vi "Receiver_Example - 2 Channel - Experiment_14.vi"() -> ()   [LabVIEW 2022 SP3]
panel:
  in  "stop":bool
  out "BER LP3":dbl
  out "BER HP3":dbl
  out "Inst. BER LP - CH1":dbl format="%#_4g"
  out "OutputHPCH0":i8[](array[numeric])
  out "BER 16QAM":dbl
  out "LP - CH0":dbl format="%#_4g"
  out "Numeric":i32
  out "HP - CH0":dbl format="%#_4g"
  out "x = 0?":bool
  out "iterationsIM":dbl
  in  "State":i32
  in  "Counter":dbl
  in  "Tab Control 3":enum32{"OFDM - 4QAM", "16QAM"}(tab)
  in  "Switch mode":bool
  in  "Tab Control":T1(tab)
  in  "USRP ControledParameters":T2={"Active Antenna"="RX2", "Gain (dB)"=10.0, "Carrier Frequency"=2400000000.0, "IQ Rate"=2000000.0, "Active channels"="0,1"} {"IQ Rate" format="%#_6p"; "Carrier Frequency" format="%#_6p"; "Gain (dB)" format="%#_6f"}
  in  "Device selection":refnum<k15>="RIO0"
  in  "Trigger level":dbl=0.01 format="%f"
  out "CH0":T3
  out "CH1":T3
  out "SIG valid? - CH1":bool
  out "SIG valid? - CH0":bool
  out "Frequency offset - CH1":dbl
  out "Frequency offset - CH0":dbl
  out "Coerced Parameters":T4={"IQ Rate"=100000.0, "Carrier  Freq."=100000.0, "Gain"=0.0} {"Gain" format="%#_6f"; "Carrier  Freq." format="%#_6p"; "IQ Rate" format="%#_6p"}
  out "Error out":errorcluster
  out "Inst. BER HP - CH0":dbl format="%#_4g"
  out "Acc. BER HP - CH0":dbl format="%#_4g"
  out "Acum. Err HP - CH0":dbl
  out "No. Bits HP - CH0":dbl
  out "Acc. BER LP - CH0":dbl format="%#_4g"
  out "Inst. BER - CH1":dbl format="%#_4g"
  out "Inst. BER LP - CH0":dbl format="%#_4g"
  out "No. Bits - CH1":dbl
  out "No. Bits LP - CH0":dbl
  out "Acum. Err - CH1":dbl
  out "Acum. Err LP - CH0":dbl
  in  "Record BER":bool
  in  "Refresh Button":bool
  out "Acc. BER - CH1":dbl format="%#_4g"
  in  "Boolean 2":bool
  in  "Expected message HP - CH0":string="Critical Dataaaaa\nCritical Dataaaaa\nCritical Dataaaaa\nCritical Dataaaaa\nCritical Dataaaaa"
  out "Expected message HP Detected CH0":string="Non Critical Data\nNon Critical Data\nNon Critical Data\nNon Critical Data\nNon Critical Data"
  in  "Boolean 3":bool
  in  "Boolean":bool
  out "Expected message HP Detected CH1":string="Non Critical Data\nNon Critical Data\nNon Critical Data\nNon Critical Data\nNon Critical Data"
  out "Expected message LP Detected CH0":string="Non Critical Data\nNon Critical Data\nNon Critical Data\nNon Critical Data\nNon Critical Data"
  in  "Expected message - CH1":string="Critical Dataaaaa\nCritical Dataaaaa\nCritical Dataaaaa\nCritical Dataaaaa\nCritical Dataaaaa"
  in  "Expected message LP - CH0":string="Non Critical Data\nNon Critical Data\nNon Critical Data\nNon Critical Data\nNon Critical Data"
  in  "Boolean 5":bool
  in  "Expected message LP - CH1":string="Non Critical Data\nNon Critical Data\nNon Critical Data\nNon Critical Data\nNon Critical Data"
  out "Expected message LP Detected CH1":string="Non Critical Data\nNon Critical Data\nNon Critical Data\nNon Critical Data\nNon Critical Data"
  in  "High-Power Window Size":dbl=15.0 format="%#_6p"
  in  "Low-Power Window Size - CH0":dbl=15.0 format="%#_6p"
  in  "Channel":bool
  in  "Expected message HP - CH0 2":string="Critical Dataaaaa\nCritical Dataaaaa\nCritical Dataaaaa\nCritical Dataaaaa\nCritical Dataaaaa\nNon Critical Data\nNon Critical Data\nNon Critical Data\nNon Critical Data\nNon Critical Data"
  in  "Tab Control 2":enum32{"1 Channel", "2 Channel"}(tab)
  in  "Save data 1 channel":bool
  out "Constellation Map 1 Channel":cdb[](graph)
  out "Low-Power BER - 1 Channel":dbl(graph)
  out "High-Power BER - 1 Channel":dbl(graph)
  out "High-Power Decoded message - 1 Channel":string
  out "Low-Power Decoded message - 1 Channel":string
  out "Low-Power Decoded message - CH0":string
  out "Decoded message - CH1":string
  out "Constellation Map 2 Channel":cluster{"Constellation":cdb[]}[](graph)
  out "Low-Power BER - 2 Channels":T5(graph)
  out "High-Power BER":T6(graph)
  out "High-Power Decoded message - CH0":string
  out "Low-Power Decoded message - CH1":string
  out "CH1 2":bool
  out "CH0 2":bool
  in  "Save data 2 channels":bool
  in  "Color Box 3":u32(colorbox)=11025761
  in  "Color Box 4":u32(colorbox)=7377308
  in  "Save data":bool
  out "Expected message  HP  Detected 2":string="Critical Dataaaaa\nCritical Dataaaaa\nCritical Dataaaaa\nCritical Dataaaaa\nCritical Dataaaaa"
  in  "Boolean 4":bool
  in  "High-Power Window Size 2":dbl=15.0 format="%#_6p"
  out "High-Power Instantaneous BER Graph 2":u8(slide) scale=0.0..100.0
  out "High-Power BER Graph 2":dbl(graph)
  out "No. Bits HP 2":dbl
  out "Acc. BER  HP 2":dbl format="%#_4g"
  out "Acum. Err HP 2":dbl
  out "Inst. BER HP 2":dbl format="%#_4g"
  in  "Expected message 2 HP 2":string="Critical Dataaaaa\nCritical Dataaaaa\nCritical Dataaaaa\nCritical Dataaaaa\nCritical Dataaaaa"
  out "High-Power Decoded Message 2":string
  in  "Record BER 2":bool
  out "Constellation Map 2":cdb[](graph)
  out "Frequency offset 2":dbl
  out "SIG valid? 2":bool
  in  "Refresh Button 2":bool
  out "Error out 2":errorcluster
  in  "error in (no error)":errorcluster
  # "OFDM Superposition Coded Receiver"
  # "Superposition coded\n(criticality-aware)"
  # "Single stream\n(criticality-agnostic)"
  # "1 Channel"
  # "2 Channel"
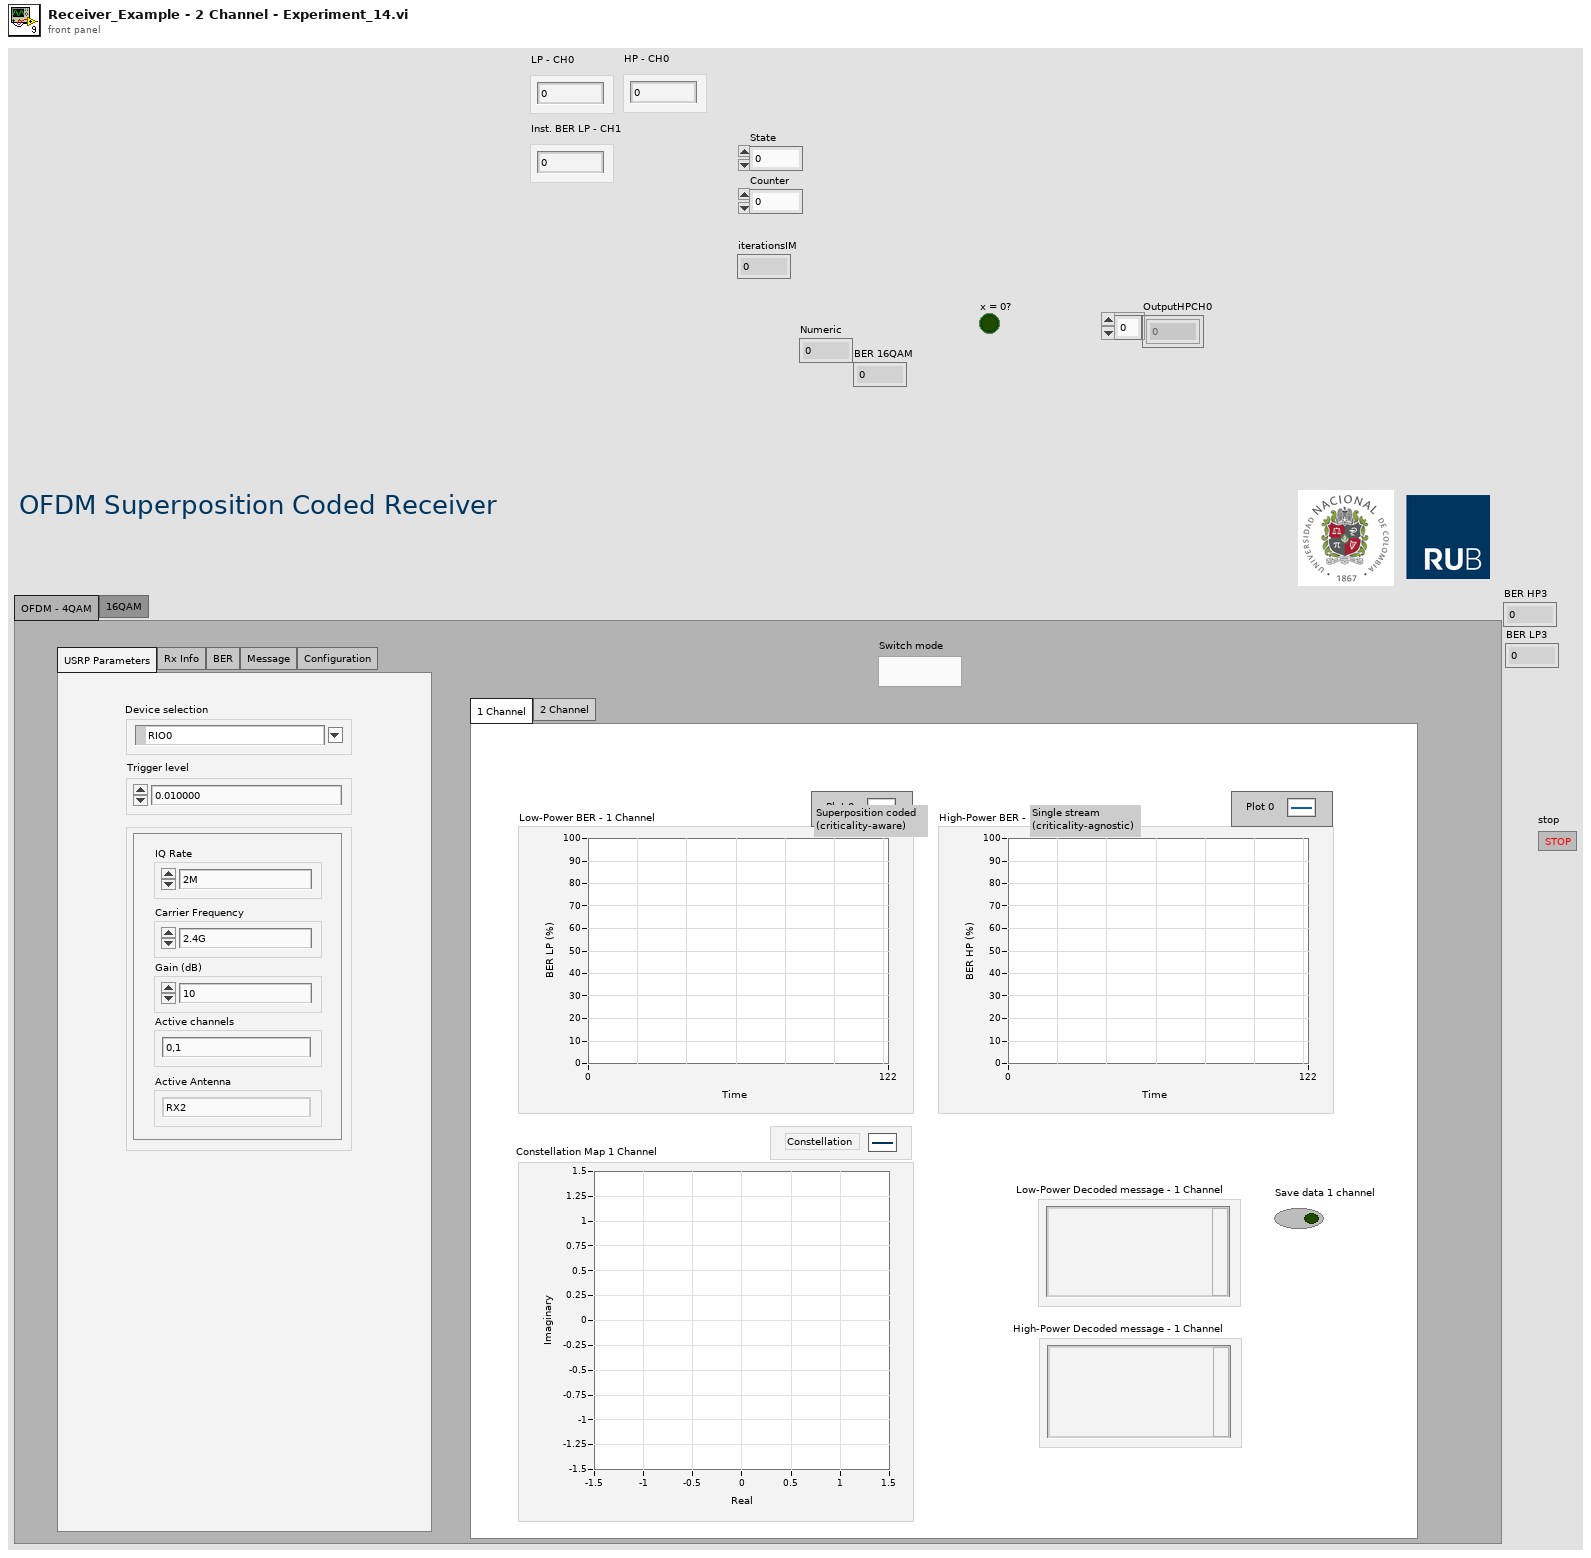
[diagram p1: front panel]
types:
  T1 = enum32{"USRP Parameters", "Rx Info", "BER", "Message", "Configuration"}
  T2 = cluster{"Active Antenna":string, "Gain (dB)":dbl, "Carrier Frequency":dbl, "IQ Rate":dbl, "Active channels":string}
  T3 = cluster{"Modulation type":enum16{"QPSK(4QAM)", "64QAM", "16QAM", "BPSK"}, "BCC rate (k/n)":enum16{"1/2", "2/3", "3/4"}}
  T4 = cluster{"IQ Rate":dbl, "Carrier  Freq.":dbl, "Gain":dbl}
  T5 = cluster{"Graph Instantaneous BER":dbl, "Graph Instantaneous BER":dbl, "Graph Instantaneous BER":dbl}
  T6 = cluster{"Graph Instantaneous BER":dbl, "Graph Instantaneous BER":dbl, "Inst. BER - CH1":dbl}
  T7 = enum16{"open", "replace", "create", "open or create", "replace or create", "replace or create with confirmation"}
  T8 = cluster{"coerced IQ rate":dbl, "coerced carrier frequency":dbl, "coerced gain":dbl}
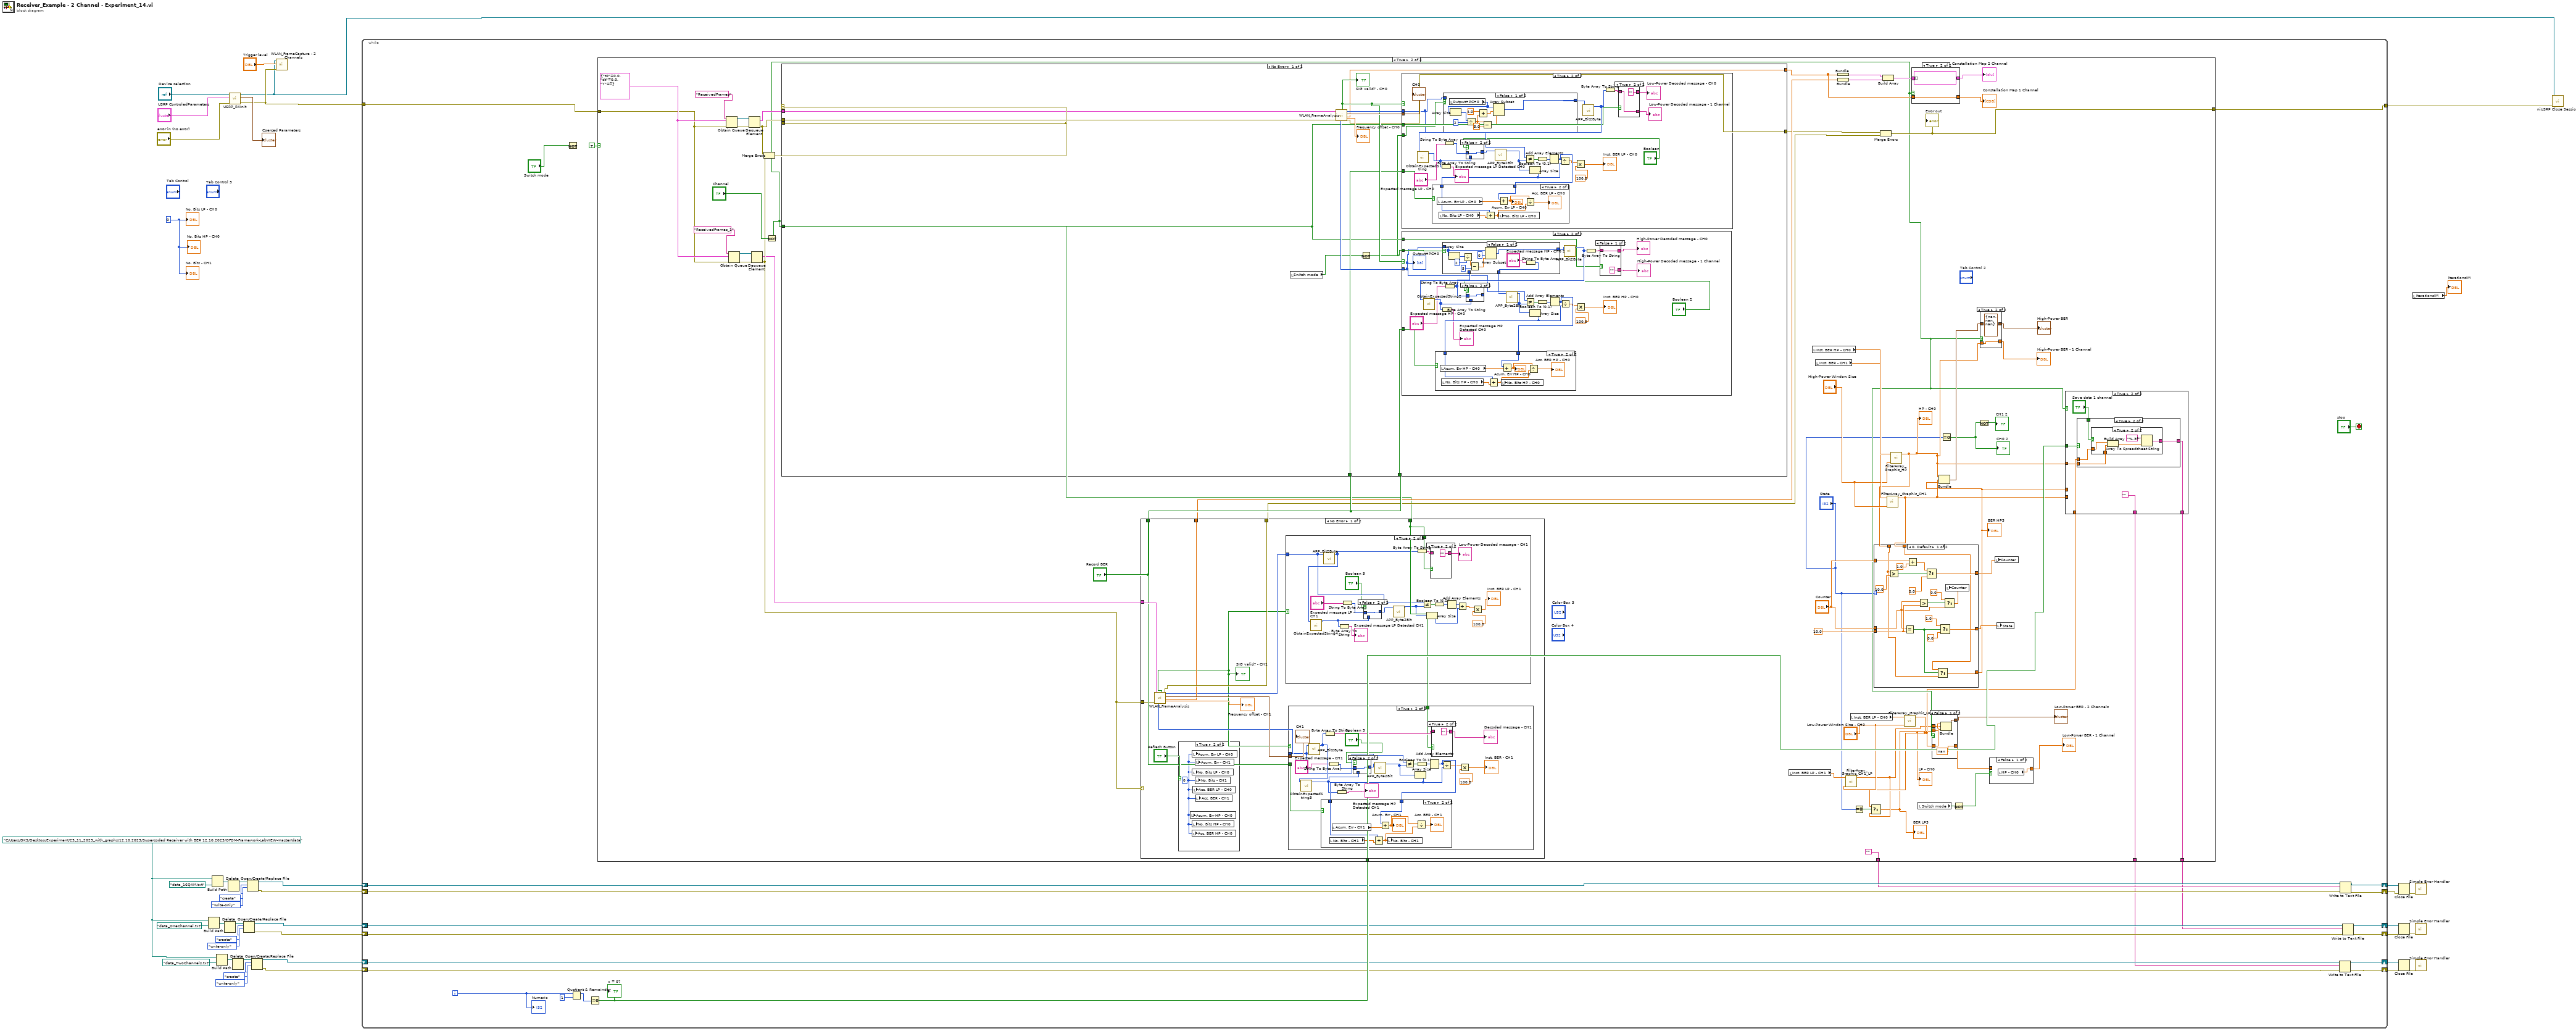
[diagram p0: block diagram]
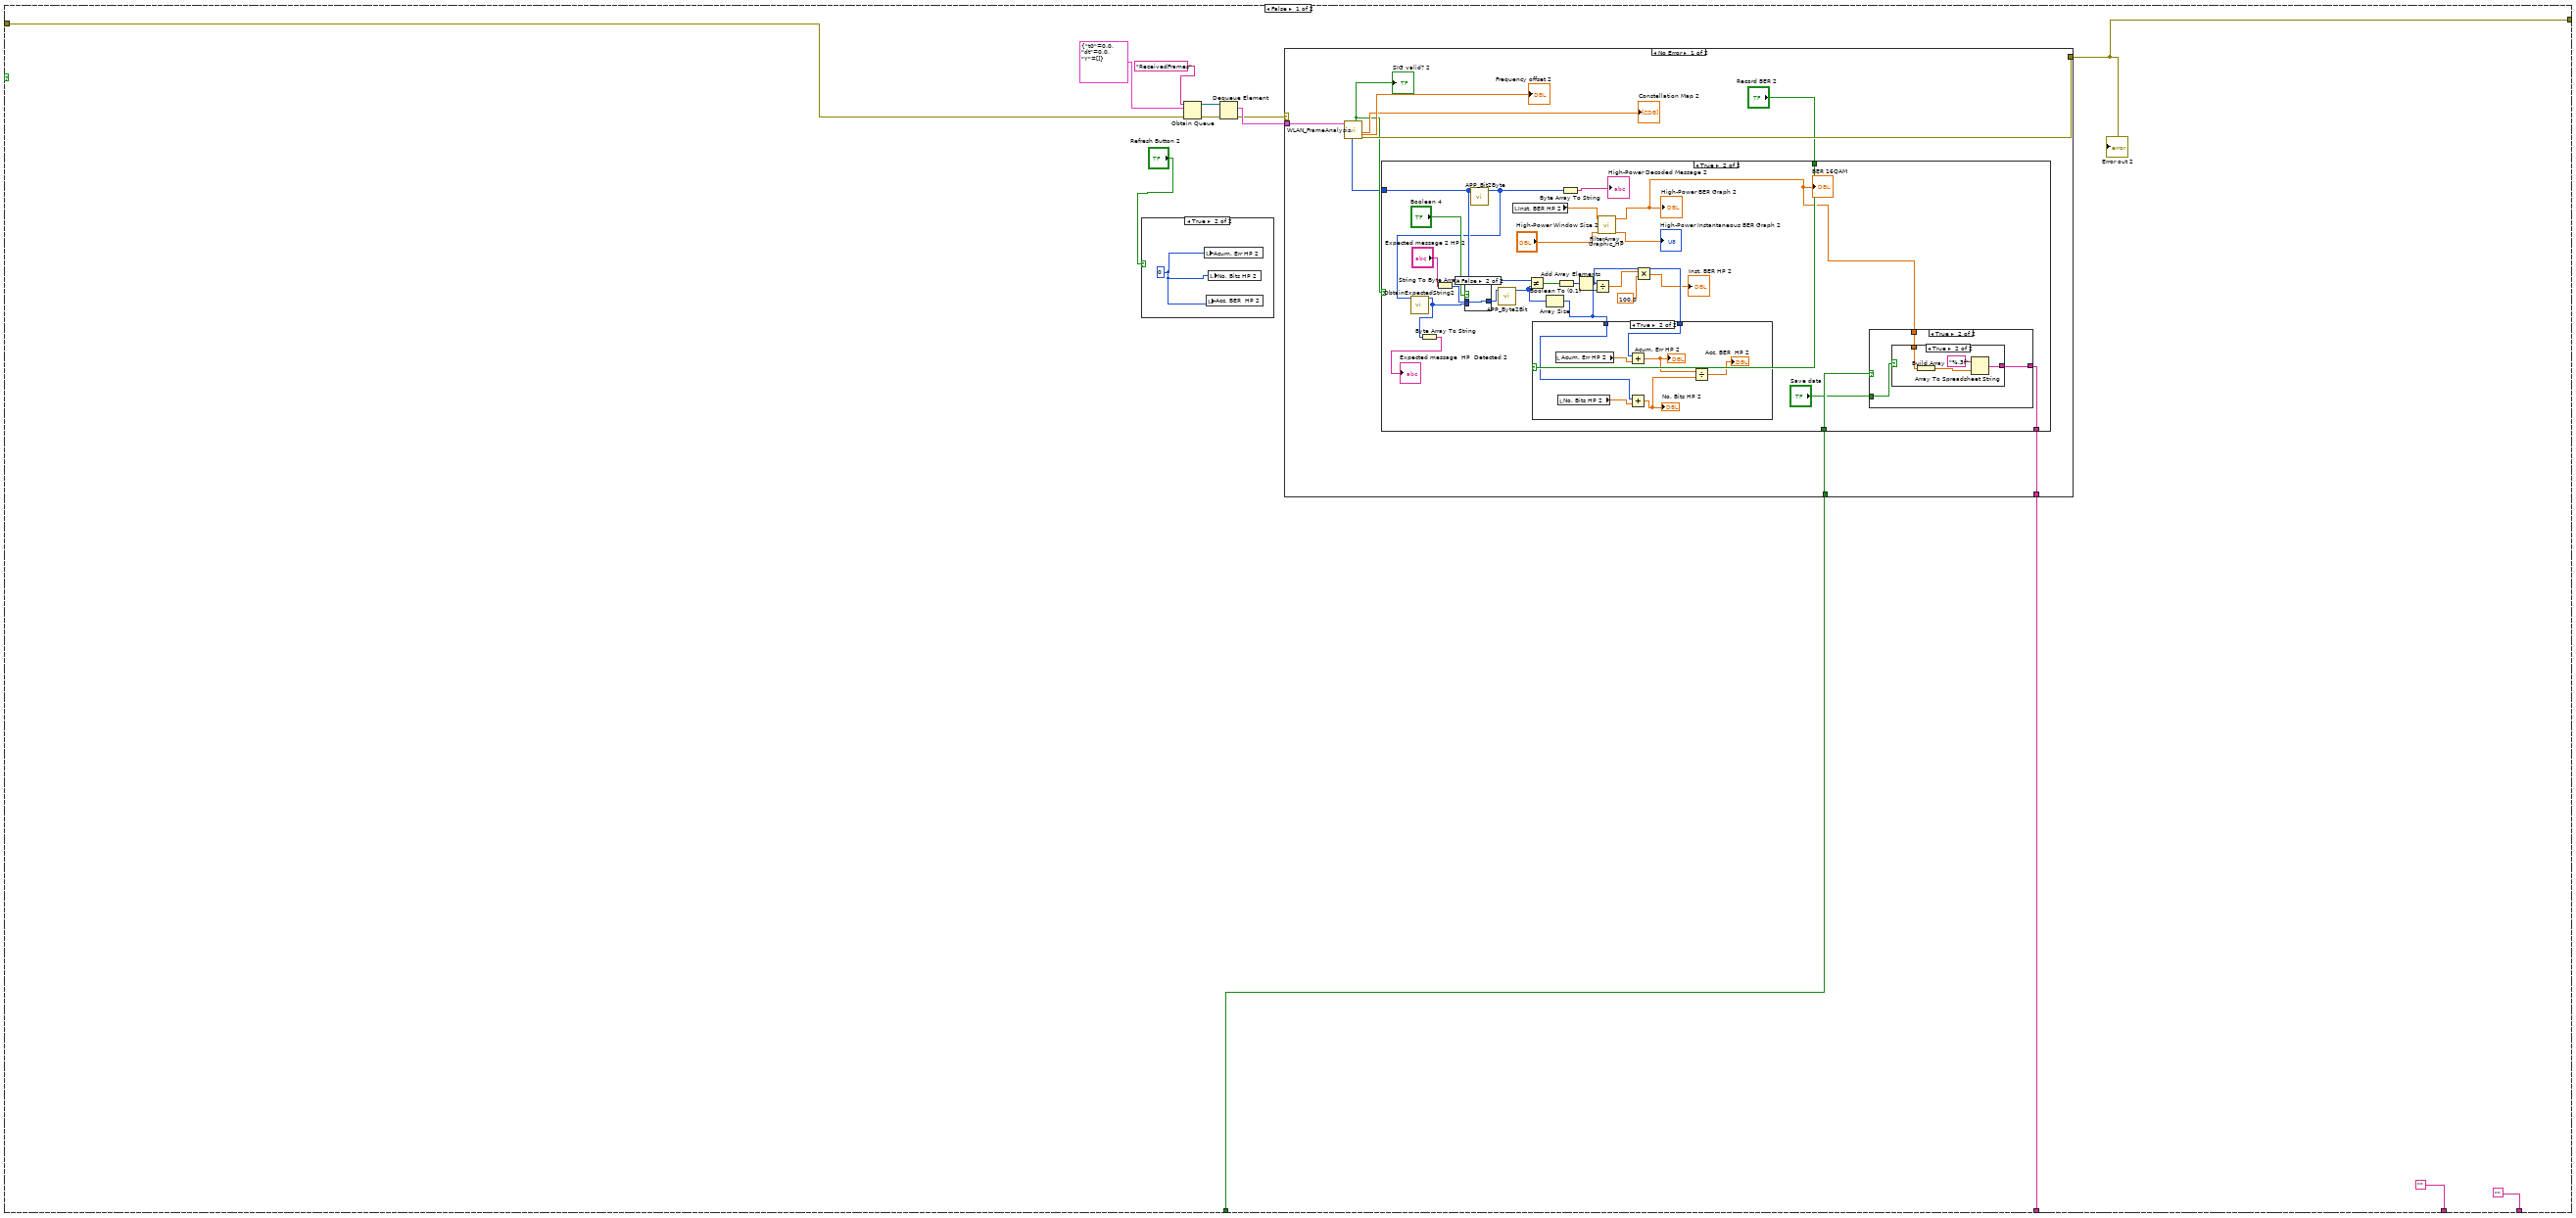
[diagram p2: hidden frame]
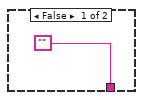
[diagram p4: hidden frame]
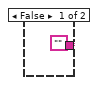
[diagram p5: hidden frame]
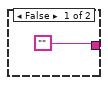
[diagram p6: hidden frame]
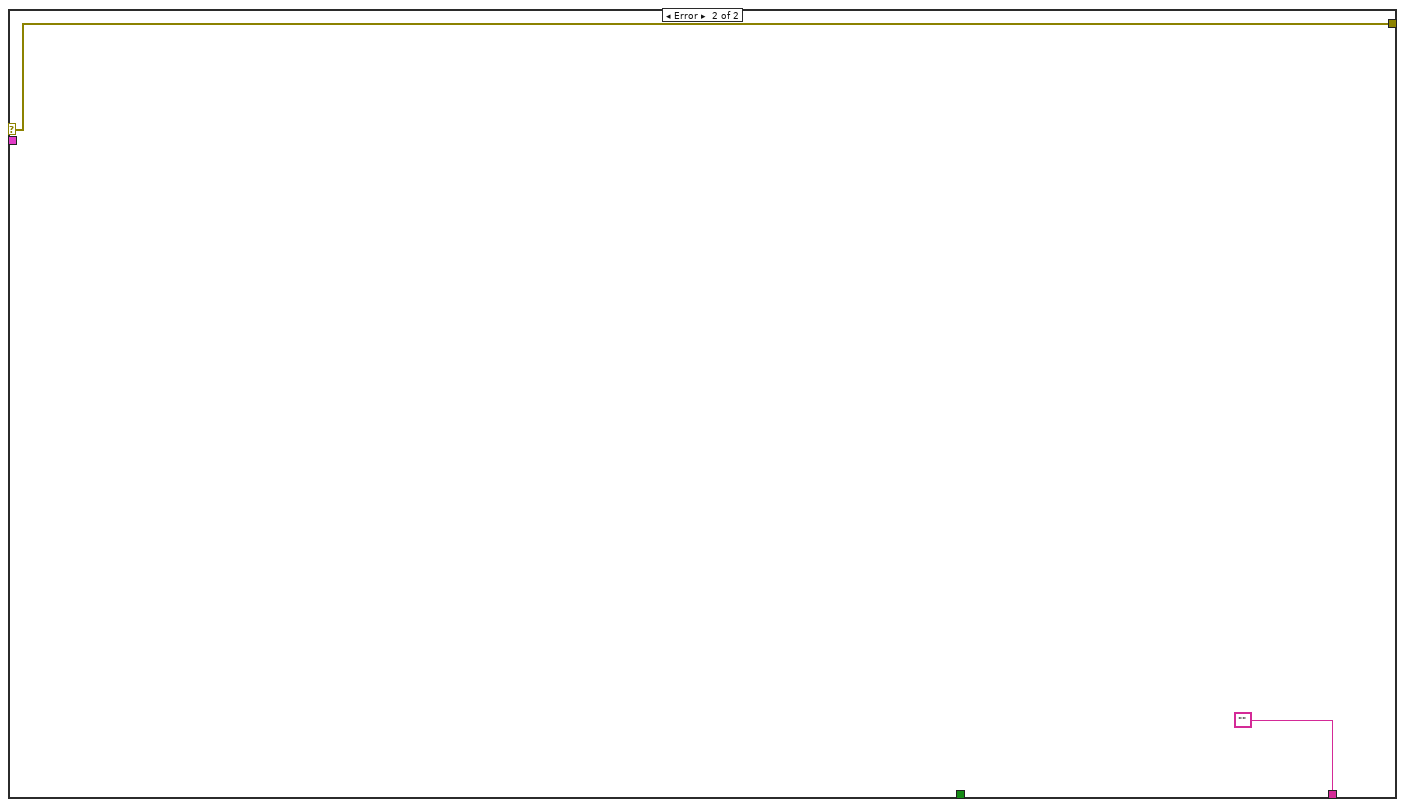
[diagram p9: hidden frame]
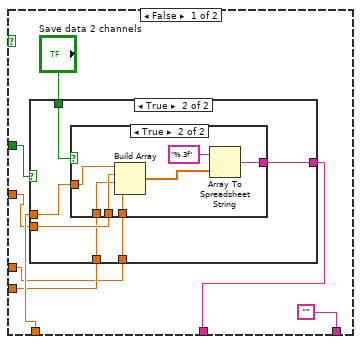
[diagram p11: hidden frame]
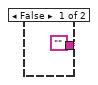
[diagram p12: hidden frame]
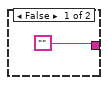
[diagram p13: hidden frame]
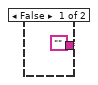
[diagram p14: hidden frame]
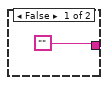
[diagram p15: hidden frame]
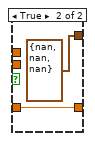
[diagram p16: hidden frame]
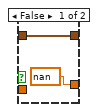
[diagram p17: hidden frame]
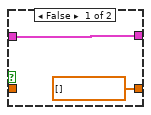
[diagram p18: hidden frame]
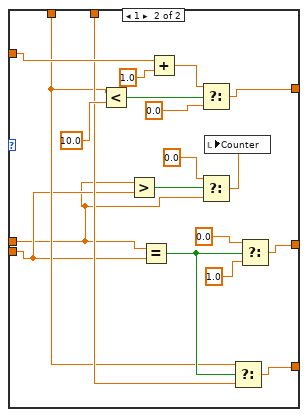
[diagram p19: hidden frame]
diagram:
  w11 = path "C:/Users/DKS/Desktop/Experiment/23_11_2023_with_graphs/12.10.2023/Supercoded Receiver with BER 12.10.2023/OFDM-Framework-LabVIEW-master/data"
  w33 = 0
  n1 = Build Path(base path=w11, name or relative path=path "data_OneChannel.txt" ("default name")) -> (appended path=w21:path)
  n2 = Build Path(base path=w11, name or relative path=path "data_16QAM.txt" ("default name")) -> (appended path=w31:path)
  n3 = Build Path(base path=w11, name or relative path=path "data_TwoChannels.txt" ("default name")) -> (appended path=w16:path)
  n4 = Delete(path (use dialog)=w21) -> (deleted path=w20:path)  [unwired: 4 in, 2 out]
  n5 = Delete(path (use dialog)=w31) -> (deleted path=w30:path)  [unwired: 4 in, 2 out]
  n6 = call "USRP_RXInit.vi"("device names"="Device selection", "USRP ControledParameters"="USRP ControledParameters", "error in (no error)"="error in (no error)") -> ("session handle out"=w36:refnum<k15>, "USRP CoercedParamters"=→"Coerced Parameters":T8, "error out"=w39:errorcluster)  [unwired: 5 in]
  n7 = Delete(path (use dialog)=w16) -> (deleted path=w15:path)  [unwired: 4 in, 2 out]
  n8 = Open/Create/Replace File(file path (use dialog)=w20, operation (0:open)=T7."create", access (0:read/write)=enum16{"read/write", "read-only", "write-only"}."write-only") -> (refnum out=w8:refnum<file>, error out=w7:errorcluster)  [unwired: 1 in, 3 out]
  n9 = Open/Create/Replace File(file path (use dialog)=w30, operation (0:open)=T7."create", access (0:read/write)=enum16{"read/write", "read-only", "write-only"}."write-only") -> (refnum out=w24:refnum<file>, error out=w25:errorcluster)  [unwired: 1 in, 3 out]
  n10 = Open/Create/Replace File(file path (use dialog)=w15, operation (0:open)=T7."create", access (0:read/write)=enum16{"read/write", "read-only", "write-only"}."write-only") -> (refnum out=w6:refnum<file>, error out=w5:errorcluster)  [unwired: 1 in, 3 out]
  n11 = call "WLAN_FrameCapture - 2 Channels.vi"("error in (no error)"=w39, "Trigger level"="Trigger level", "session handle"=w36) -> ()  [unwired: 8 in]
  n12 = while {
    tunnel: w39 -> [w65]
    tunnel: [w64] -> w37
    shift-right: [w60] -> w23
    shift-left: w25 -> [w58]
    shift-right: [w59] -> w22
    shift-left: w24 -> [w57]
    shift-right: [w54] -> w4
    shift-left: w8 -> [w55]
    shift-right: [w52] -> w3
    shift-left: w7 -> [w53]
    shift-right: [w48] -> w2
    shift-left: w6 -> [w51]
    shift-right: [w49] -> w1
    shift-left: w5 -> [w50]
    i -> [w45]
    stop <- "stop" stop-if-true
    n13 = Not(x="Switch mode") -> ()  [unwired: 1 out]
    n14 = Quotient & Remainder(x=w45, y=1) -> (x-y*floor(x/y)=w62:i32)  [unwired: 1 out]
    n15 = Equal To 0?(x=w62) -> (x = 0?=w61:bool)
    "x = 0?" <- w61
    n16 = case shown="True" TRUE {
      tunnel: w65 -> [w71 w157]
      tunnel: [w70 w156] -> w64
      tunnel: w61 -> [w69 w152]
      tunnel: [w68 ""] -> w56
      tunnel: ["" w151] -> w47
      tunnel: ["" w149] -> w46
      frame False {
        n17 = case shown="True" "Refresh Button 2" {
          frame False {
          }
          frame True {
            w79 = 0
            n18 = local write "Acum. Err HP 2"(w79) -> ()
            n19 = local write "Acc. BER  HP 2"(w79) -> ()
            n20 = local write "No. Bits HP 2"(w79) -> ()
          }
        }
        n21 = Obtain Queue(name (unnamed)="ReceivedFrames", element data type=cluster{"t0":dbl, "dt":dbl, "Y":cdb[]} {"t0"=0.0, "dt"=0.0, "Y"=[]} ("data"), error in (no error)=w71) -> (queue out=w72:refnum<queue>, error out=w75:errorcluster)  [unwired: 2 in, 1 out]
        n22 = Dequeue Element(queue=w72, error in (no error)=w75) -> (element=w74:cluster{"t0":dbl, "dt":dbl, "Y":cdb[]}, error out=w73:errorcluster)  [unwired: 1 in, 2 out]
        n23 = case shown="No Error" w73 {
          selector: w73 -> [_ w134]
          tunnel: w74 -> [w87 _]
          tunnel: [w88 w134] -> w70
          tunnel: w69 -> [w81 _]
          tunnel: [w80 ""] -> w68
          frame No Error {
            n24 = call "WLAN_FrameAnalysis.vi"("input cluster"=w87) -> ("error out"=w88:errorcluster, "Constellation"=→"Constellation Map 2":cdb[], "Frequency offset"=→"Frequency offset 2":dbl, "SIG valid?"=w83:bool, "outputbitsHP"=w82:i8[])  [unwired: 4 in, 2 out]
            "SIG valid? 2" <- w83
            n25 = case shown="True" w83 {
              tunnel: "Record BER 2" -> [_ w108]
              tunnel: w82 -> [_ w103]
              tunnel: w81 -> [_ w93]
              tunnel: ["" w91] -> w80
              frame False {
              }
              frame True {
                n26 = String To Byte Array(string="Expected message 2 HP 2") -> (unsigned byte array=w101:u8[])
                n27 = call "APP_Bit2Byte.vi"("input bit stream"=w103) -> ("output byte stream"=w97:u8[])  [unwired: 10 in]
                n28 = call "ObtainExpectedString2.vi"("Array"=w97) -> ("detectedMessage"=w99:i8[])  [unwired: 9 in]
                n29 = Byte Array To String(unsigned byte array=w99) -> (string=→"Expected message  HP  Detected 2":string)
                n30 = case shown="False" "Boolean 4" {
                  tunnel: [w124 w125] -> w102
                  tunnel: w101 -> [_ w125]
                  tunnel: w99 -> [w124 _]
                  frame True {
                  }
                  frame False {
                  }
                }
                n31 = call "APP_Byte2Bit.vi"("input byte stream"=w102) -> ("output bit stream"=w104:i8[])  [unwired: 10 in]
                n32 = local read "Inst. BER HP 2"() -> (w107:dbl)
                n33 = Not Equal?(x=w103, y=w104) -> (x != y?=w112:bool[])
                n34 = Array Size(array=w104) -> (size(s)=w109:i32)
                n35 = Boolean To (0,1)(Boolean=w112) -> (0, 1=w111:i16[])
                n36 = Byte Array To String(unsigned byte array=w97) -> (string=→"High-Power Decoded Message 2":string)
                n37 = Add Array Elements(numeric array=w111) -> (sum=w110:i16)
                n38 = case shown="True" w108 {
                  tunnel: w110 -> [_ w131]
                  tunnel: w109 -> [_ w126]
                  frame False {
                  }
                  frame True {
                    n39 = local read "Acum. Err HP 2"() -> (w132:dbl)
                    n40 = local read "No. Bits HP 2"() -> (w128:dbl)
                    n41 = Add(x=w131, y=w132) -> (x+y=w130:dbl)
                    "Acum. Err HP 2" <- w130
                    n42 = Add(x=w126, y=w128) -> (x+y=w127:dbl)
                    "No. Bits HP 2" <- w127
                    n43 = Divide(x=w130, y=w127) -> (x/y=→"Acc. BER  HP 2":dbl)
                  }
                }
                n44 = Divide(x=w110, y=w109) -> (x/y=w96:dbl)
                n45 = call "FilterArray_Graphic_HP.vi"("Window Size"="High-Power Window Size 2", "Instantaneous BER"=w107) -> ("Slide Bar"=→"High-Power Instantaneous BER Graph 2":dbl, "Graph Instantaneous BER"=w90:dbl)  [unwired: 4 in]
                "High-Power BER Graph 2" <- w90
                "BER 16QAM" <- w90
                n46 = Multiply(x=w96, y=100.0) -> (x*y=→"Inst. BER HP 2":dbl)
                n47 = case shown="True" w93 {
                  tunnel: ["" w118] -> w91
                  tunnel: w90 -> [_ w117]
                  tunnel: "Save data" -> [_ w116]
                  frame False {
                  }
                  frame True {
                    n48 = case shown="True" w116 {
                      tunnel: ["" w121] -> w118
                      tunnel: w117 -> [_ w120]
                      frame False {
                      }
                      frame True {
                        n49 = Build Array(w120) -> (w123:dbl[])
                        n50 = Array To Spreadsheet String(array=w123, 3:"%.3f") -> (spreadsheet string=w121:string)  [unwired: 1 out]
                      }
                    }
                  }
                }
              }
            }
          }
          frame Error {
          }
        }
        "Error out 2" <- w70
      }
      frame True {
        w192 = cluster{"t0":dbl, "dt":dbl, "Y":cdb[]} {"t0"=0.0, "dt"=0.0, "Y"=[]} ("data")
        n51 = Obtain Queue(name (unnamed)="ReceivedFrames", element data type=w192, error in (no error)=w157) -> (queue out=w158:refnum<queue>, error out=w160:errorcluster)  [unwired: 2 in, 1 out]
        n52 = Obtain Queue(name (unnamed)="ReceivedFrames_1", element data type=w192, error in (no error)=w157) -> (queue out=w162:refnum<queue>, error out=w163:errorcluster)  [unwired: 2 in, 1 out]
        n53 = Dequeue Element(queue=w158, error in (no error)=w160) -> (element=w159:cluster{"t0":dbl, "dt":dbl, "Y":cdb[]}, error out=w166:errorcluster)  [unwired: 1 in, 2 out]
        n54 = Dequeue Element(queue=w162, error in (no error)=w163) -> (element=w168:cluster{"t0":dbl, "dt":dbl, "Y":cdb[]}, error out=w172:errorcluster)  [unwired: 1 in, 2 out]
        n55 = Merge Errors(w166, w172) -> (w165:errorcluster)
        n56 = Not(x="Channel") -> (.not. x?=w153:bool)
        n57 = case shown="No Error" w165 {
          tunnel: w159 -> [w368 _]
          tunnel: w165 -> [_ w468]
          tunnel: w166 -> [w365 _]
          tunnel: [w364 dbl[] []] -> w183
          tunnel: [w363 w468] -> w169
          tunnel: "Record BER" -> [w362 _]
          tunnel: "Record BER" -> [w361 _]
          tunnel: w153 -> [w360 _]
          frame No Error {
            n58 = local read "Switch mode"() -> (w359:bool)
            n59 = call "WLAN_FrameAnalysis.vi"("error in (no error)"=w365, "input cluster"=w368) -> ("error out"=w363:errorcluster, "Constellation"=w364:cdb[], "Modulation parameter"=w369:T3, "output bits"=w370:i8[], "Frequency offset"=→"Frequency offset - CH0":dbl, "SIG valid?"=w366:bool, "outputbitsHP"=w367:i8[])  [unwired: 3 in]
            "SIG valid? - CH0" <- w366
            n60 = Not(x=w359) -> (.not. x?=w358:bool)
            n61 = case shown="True" w366 {
              tunnel: w370 -> [_ w423]
              tunnel: w369 -> [_ w443]
              tunnel: w361 -> [_ w440]
              tunnel: w360 -> [_ w426]
              tunnel: w358 -> [_ w424]
              frame False {
              }
              frame True {
                n62 = case shown="False" w424 {
                  tunnel: w423 -> [_ w453]
                  tunnel: [w451 w453] -> w425
                  frame False {
                    n63 = local read "OutputHPCH0"() -> (w450:i8[])
                    n64 = Array Size(array=w450) -> (size(s)=w449:i32)
                    n65 = Divide(x=w449, y=2) -> (x/y=w446:dbl)
                    n66 = Add(x=4.0, y=w446) -> (x+y=w448:dbl)
                    n67 = Subtract(x=w446, y=5.0) -> (x-y=w444:dbl)
                    n68 = Array Subset(array=w450, index=w448, length=w444) -> (w451:i8[])
                  }
                  frame True {
                  }
                }
                n69 = String To Byte Array(string="Expected message LP - CH0") -> (unsigned byte array=w433:u8[])
                n70 = call "APP_Bit2Byte.vi"("input bit stream"=w425) -> ("output byte stream"=w432:u8[])  [unwired: 10 in]
                n71 = call "ObtainExpectedString.vi"("Array"=w432) -> ("detectedMessage"=w431:i8[])  [unwired: 9 in]
                n72 = Byte Array To String(unsigned byte array=w431) -> (string=→"Expected message LP Detected CH0":string)
                n73 = case shown="False" "Boolean" {
                  tunnel: [w458 w459] -> w435
                  tunnel: w433 -> [_ w459]
                  tunnel: w431 -> [w458 _]
                  frame True {
                  }
                  frame False {
                  }
                }
                n74 = call "APP_Byte2Bit.vi"("input byte stream"=w435) -> ("output bit stream"=w434:i8[])  [unwired: 10 in]
                n75 = Not Equal?(x=w423, y=w434) -> (x != y?=w441:bool[])
                n76 = Array Size(array=w434) -> (size(s)=w439:i32)
                n77 = Boolean To (0,1)(Boolean=w441) -> (0, 1=w442:i16[])
                n78 = Add Array Elements(numeric array=w442) -> (sum=w438:i16)
                n79 = case shown="True" w440 {
                  tunnel: w439 -> [_ w465]
                  tunnel: w438 -> [_ w463]
                  frame False {
                  }
                  frame True {
                    n80 = local read "Acum. Err LP - CH0"() -> (w464:dbl)
                    n81 = local read "No. Bits LP - CH0"() -> (w466:dbl)
                    n82 = Add(x=w465, y=w466) -> (x+y=w462:dbl)
                    n83 = Add(x=w463, y=w464) -> (x+y=w461:dbl)
                    "Acum. Err LP - CH0" <- w461
                    n84 = local write "No. Bits LP - CH0"(w462) -> ()
                    n85 = Divide(x=w461, y=w462) -> (x/y=→"Acc. BER LP - CH0":dbl)
                  }
                }
                n86 = Divide(x=w438, y=w439) -> (x/y=w437:dbl)
                n87 = Multiply(x=w437, y=100.0) -> (x*y=→"Inst. BER LP - CH0":dbl)
                n88 = Byte Array To String(unsigned byte array=w432) -> (string=w429:string)
                n89 = case shown="True" w426 {
                  tunnel: w429 -> [w455 w457]
                  tunnel: ["" ("string") w457] -> w428
                  tunnel: [w455 "" ("string")] -> w427
                  frame False {
                  }
                  frame True {
                  }
                }
                "Low-Power Decoded message - CH0" <- w427
                "Low-Power Decoded message - 1 Channel" <- w428
                "CH0" <- w443
              }
            }
            n90 = case shown="True" w366 {
              tunnel: w367 -> [_ w376]
              tunnel: w362 -> [_ w392]
              tunnel: w360 -> [_ w381]
              tunnel: w358 -> [_ w379]
              frame False {
              }
              frame True {
                n91 = String To Byte Array(string="Expected message HP - CH0") -> (unsigned byte array=w378:u8[])
                n92 = case shown="False" w379 {
                  tunnel: w376 -> [w402 w406]
                  tunnel: [w403 w406] -> w380
                  tunnel: [w395 w405] -> w375
                  tunnel: w378 -> [_ w405]
                  frame False {
                    n93 = Array Size(array=w402) -> (size(s)=w399:i32)
                    n94 = Divide(x=w399, y=2) -> (x/y=w398:dbl)
                    n95 = Subtract(x=w398, y=5) -> (x-y=w400:dbl)
                    n96 = Array Subset(array=w402, index=0, length=w400) -> (w403:i8[])
                    n97 = String To Byte Array(string="Expected message HP - CH0 2") -> (unsigned byte array=w395:u8[])
                  }
                  frame True {
                  }
                }
                n98 = call "APP_Byte2Bit.vi"("input byte stream"=w375) -> ("output bit stream"=w377:i8[])  [unwired: 10 in]
                n99 = Not Equal?(x=w376, y=w377) -> (x != y?=w393:bool[])
                n100 = Array Size(array=w377) -> (size(s)=w391:i32)
                n101 = Boolean To (0,1)(Boolean=w393) -> (0, 1=w394:i16[])
                n102 = Add Array Elements(numeric array=w394) -> (sum=w390:i16)
                n103 = case shown="True" w392 {
                  tunnel: w391 -> [_ w418]
                  tunnel: w390 -> [_ w416]
                  frame False {
                  }
                  frame True {
                    n104 = local read "Acum. Err HP - CH0"() -> (w417:dbl)
                    n105 = local read "No. Bits HP - CH0"() -> (w419:dbl)
                    n106 = Add(x=w418, y=w419) -> (x+y=w415:dbl)
                    n107 = local write "No. Bits HP - CH0"(w415) -> ()
                    n108 = Add(x=w416, y=w417) -> (x+y=w414:dbl)
                    "Acum. Err HP - CH0" <- w414
                    n109 = Divide(x=w414, y=w415) -> (x/y=→"Acc. BER HP - CH0":dbl)
                  }
                }
                n110 = Divide(x=w390, y=w391) -> (x/y=w389:dbl)
                n111 = call "APP_Bit2Byte.vi"("input bit stream"=w380) -> ("output byte stream"=w387:u8[])  [unwired: 10 in]
                n112 = call "ObtainExpectedString2.vi"("Array"=w387) -> ("detectedMessage"=w386:i8[])  [unwired: 9 in]
                n113 = Byte Array To String(unsigned byte array=w386) -> (string=→"Expected message HP Detected CH0":string)
                n114 = case shown="False" "Boolean 2" {
                  tunnel: [w411 w412] -> _
                  tunnel: w378 -> [_ w412]
                  tunnel: w386 -> [w411 _]
                  frame True {
                  }
                  frame False {
                  }
                }
                n115 = Multiply(x=w389, y=100.0) -> (x*y=→"Inst. BER HP - CH0":dbl)
                n116 = Byte Array To String(unsigned byte array=w387) -> (string=w382:string)
                n117 = case shown="False" w381 {
                  tunnel: w382 -> [w408 w410]
                  tunnel: ["" ("string") w410] -> w383
                  tunnel: [w408 "" ("string")] -> w384
                  frame False {
                  }
                  frame True {
                  }
                }
                "High-Power Decoded message - CH0" <- w384
                "High-Power Decoded message - 1 Channel" <- w383
                "OutputHPCH0" <- w376
              }
            }
          }
          frame Error {
          }
        }
        n118 = case shown="No Error" w172 {
          tunnel: w168 -> [w295 _]
          tunnel: "Record BER" -> [w294 _]
          tunnel: [w293 w357] -> w170
          tunnel: [w292 dbl[] []] -> w171
          tunnel: w172 -> [w291 w357]
          tunnel: w153 -> [w288 _]
          frame No Error {
            n119 = call "WLAN_FrameAnalysis.vi"("error in (no error)"=w291, "input cluster"=w295) -> ("error out"=w293:errorcluster, "Constellation"=w292:cdb[], "Modulation parameter"=w298:T3, "output bits"=w290:i8[], "Frequency offset"=→"Frequency offset - CH1":dbl, "SIG valid?"=w289:bool, "outputbitsHP"=w296:i8[])  [unwired: 3 in]
            "SIG valid? - CH1" <- w289
            n120 = case shown="True" "Refresh Button" {
              frame False {
              }
              frame True {
                w323 = 0
                n121 = local write "Acum. Err HP - CH0"(w323) -> ()
                n122 = local write "Acc. BER HP - CH0"(w323) -> ()
                n123 = local write "Acum. Err LP - CH0"(w323) -> ()
                n124 = local write "No. Bits LP - CH0"(w323) -> ()
                n125 = local write "No. Bits HP - CH0"(w323) -> ()
                n126 = local write "Acc. BER LP - CH0"(w323) -> ()
                n127 = local write "Acum. Err - CH1"(w323) -> ()
                n128 = local write "No. Bits - CH1"(w323) -> ()
                n129 = local write "Acc. BER - CH1"(w323) -> ()
              }
            }
            n130 = case shown="True" w289 {
              tunnel: w290 -> [_ w301]
              tunnel: w288 -> [_ w316]
              frame False {
              }
              frame True {
                n131 = call "APP_Bit2Byte.vi"("input bit stream"=w301) -> ("output byte stream"=w311:u8[])  [unwired: 10 in]
                n132 = call "ObtainExpectedString4.vi"("Array"=w311) -> ("detectedMessage"=w312:i8[])  [unwired: 9 in]
                n133 = Byte Array To String(unsigned byte array=w312) -> (string=→"Expected message LP Detected CH1":string)
                n134 = String To Byte Array(string="Expected message LP - CH1") -> (unsigned byte array=w315:u8[])
                n135 = case shown="False" "Boolean 5" {
                  tunnel: [w319 w320] -> w310
                  tunnel: w315 -> [_ w320]
                  tunnel: w312 -> [w319 _]
                  frame True {
                  }
                  frame False {
                  }
                }
                n136 = call "APP_Byte2Bit.vi"("input byte stream"=w310) -> ("output bit stream"=w302:i8[])  [unwired: 10 in]
                n137 = Byte Array To String(unsigned byte array=w311) -> (string=w318:string)
                n138 = Not Equal?(x=w301, y=w302) -> (x != y?=w308:bool[])
                n139 = Array Size(array=w302) -> (size(s)=w307:i32)
                n140 = case shown="True" w316 {
                  tunnel: w318 -> [w321 _]
                  tunnel: [w321 "" ("string")] -> w317
                  frame False {
                  }
                  frame True {
                  }
                }
                "Low-Power Decoded message - CH1" <- w317
                n141 = Boolean To (0,1)(Boolean=w308) -> (0, 1=w309:i16[])
                n142 = Add Array Elements(numeric array=w309) -> (sum=w306:i16)
                n143 = Divide(x=w306, y=w307) -> (x/y=w305:dbl)
                n144 = Multiply(x=w305, y=100.0) -> (x*y=→"Inst. BER LP - CH1":dbl)
              }
            }
            n145 = case shown="True" w289 {
              tunnel: w296 -> [_ w332]
              tunnel: w298 -> [_ w344]
              tunnel: w294 -> [_ w330]
              tunnel: w288 -> [_ w327]
              frame False {
              }
              frame True {
                n146 = call "APP_Bit2Byte.vi"("input bit stream"=w332) -> ("output byte stream"=w334:u8[])  [unwired: 10 in]
                n147 = call "ObtainExpectedString3.vi"("Array"=w334) -> ("detectedMessage"=w333:i8[])  [unwired: 9 in]
                n148 = Byte Array To String(unsigned byte array=w334) -> (string=w328:string)
                n149 = String To Byte Array(string="Expected message - CH1") -> (unsigned byte array=w335:u8[])
                n150 = Byte Array To String(unsigned byte array=w333) -> (string=→"Expected message HP Detected CH1":string)
                n151 = case shown="False" "Boolean 3" {
                  tunnel: [w347 w348] -> w337
                  tunnel: w335 -> [_ w348]
                  tunnel: w333 -> [w347 _]
                  frame True {
                  }
                  frame False {
                  }
                }
                n152 = call "APP_Byte2Bit.vi"("input byte stream"=w337) -> ("output bit stream"=w336:i8[])  [unwired: 10 in]
                n153 = Not Equal?(x=w332, y=w336) -> (x != y?=w342:bool[])
                n154 = Array Size(array=w336) -> (size(s)=w341:i32)
                n155 = Boolean To (0,1)(Boolean=w342) -> (0, 1=w343:i16[])
                n156 = Add Array Elements(numeric array=w343) -> (sum=w340:i16)
                n157 = case shown="True" w330 {
                  tunnel: w341 -> [_ w354]
                  tunnel: w340 -> [_ w352]
                  frame False {
                  }
                  frame True {
                    n158 = local read "No. Bits - CH1"() -> (w355:dbl)
                    n159 = local read "Acum. Err - CH1"() -> (w353:dbl)
                    n160 = Add(x=w354, y=w355) -> (x+y=w351:dbl)
                    n161 = Add(x=w352, y=w353) -> (x+y=w350:dbl)
                    "Acum. Err - CH1" <- w350
                    n162 = local write "No. Bits - CH1"(w351) -> ()
                    n163 = Divide(x=w350, y=w351) -> (x/y=→"Acc. BER - CH1":dbl)
                  }
                }
                n164 = case shown="True" w327 {
                  tunnel: w328 -> [w345 _]
                  tunnel: [w345 "" ("string")] -> w329
                  frame False {
                  }
                  frame True {
                  }
                }
                "Decoded message - CH1" <- w329
                n165 = Divide(x=w340, y=w341) -> (x/y=w338:dbl)
                n166 = Multiply(x=w338, y=100.0) -> (x*y=→"Inst. BER - CH1":dbl)
                "CH1" <- w344
              }
            }
          }
          frame Error {
          }
        }
        n167 = local read "Inst. BER LP - CH1"() -> (w141:dbl)
        n168 = local read "Inst. BER HP - CH0"() -> (w188:dbl)
        n169 = local read "Inst. BER - CH1"() -> (w179:dbl)
        n170 = Bundle("Constellation"=w183) -> (w182:cluster{"Constellation":cdb[]})  [unwired: 1 in]
        n171 = Bundle("Constellation"=w171) -> (w167:cluster{"Constellation":cdb[]})  [unwired: 1 in]
        n172 = call "FilterArray_Graphic_CH1_LP.vi"("Window Size"="Low-Power Window Size - CH0", "Instantaneous BER"=w141) -> ("Graph Instantaneous BER"=w136:dbl)  [unwired: 4 in, 1 out]
        n173 = local read "Inst. BER LP - CH0"() -> (w154:dbl)
        n174 = Equal To 0?(x="State") -> (x = 0?=w139:bool)
        n175 = Merge Errors(w169, w170) -> (w156:errorcluster)
        "Error out" <- w156
        n176 = Build Array(w182, w167) -> (w185:cluster{"Constellation":cdb[]}[])
        n177 = call "FilterArray_Graphic_CH1.vi"("Window Size"="High-Power Window Size", "Instantaneous BER"=w179) -> ("Graph Instantaneous BER"=w150:dbl)  [unwired: 4 in, 1 out]
        n178 = call "FilterArray_Graphic_HP.vi"("Window Size"="High-Power Window Size", "Instantaneous BER"=w188) -> ("Graph Instantaneous BER"=w147:dbl)  [unwired: 4 in, 1 out]
        "HP - CH0" <- w147
        n179 = case shown="0, Default" "State" {
          tunnel: "Counter" -> [w256 w276]
          tunnel: [w263 w279] -> w175
          tunnel: "Counter" -> [w251 w269]
          tunnel: [w260 w278] -> w176
          tunnel: [w258 w277] -> w148
          tunnel: w147 -> [w257 w274]
          tunnel: w150 -> [w255 w275]
          tunnel: 10.0 ("y") -> [w254 w270]
          frame 0, Default {
            n180 = Greater?(x=w257, y=10.0) -> (0:w264:bool)
            n181 = Equal?(x=w251, y=w254) -> (x = y?=w259:bool)
            n182 = Add(x=w256, y=1.0) -> (x+y=w266:dbl)
            n183 = Greater?(x=w251, y=w254) -> (0:w253:bool)
            n184 = Select(t=w266, s=w264, f=0.0) -> (s? t:f=w263:dbl)
            n185 = Select(t=w255, s=w259, f=w257) -> (s? t:f=w258:dbl)
            n186 = Select(t=1.0, s=w259, f=0.0) -> (s? t:f=w260:dbl)
            n187 = Select(t=0.0, s=w253, f=w251) -> (s? t:f=w250:dbl)
            n188 = local write "Counter"(w250) -> ()
          }
          frame 1 {
            n189 = Less?(x=w274, y=10.0) -> (x < y?=w280:bool)
            n190 = Greater?(x=w269, y=w270) -> (0:w272:bool)
            n191 = Equal?(x=w269, y=w270) -> (x = y?=w282:bool)
            n192 = Add(x=w276, y=1.0) -> (x+y=w286:dbl)
            n193 = Select(t=w286, s=w280, f=0.0) -> (s? t:f=w279:dbl)
            n194 = Select(t=0.0, s=w272, f=w269) -> (s? t:f=w273:dbl)
            n195 = local write "Counter"(w273) -> ()
            n196 = Select(t=w274, s=w282, f=w275) -> (s? t:f=w277:dbl)
            n197 = Select(t=0.0, s=w282, f=1.0) -> (s? t:f=w278:dbl)
          }
        }
        "BER HP3" <- w148
        n198 = call "FilterArray_Graphic_LP.vi"("Window Size"="Low-Power Window Size - CH0", "Instantaneous BER"=w154) -> ("Graph Instantaneous BER"=w137:dbl)  [unwired: 4 in, 1 out]
        "LP - CH0" <- w137
        n199 = Select(t=w137, s=w139, f=w136) -> (s? t:f=w135:dbl)
        "BER LP3" <- w135
        n200 = case shown="True" w153 {
          tunnel: [cdb[] [] ("Constellation") w249] -> w184
          tunnel: w183 -> [_ w249]
          tunnel: w185 -> [w247 _]
          tunnel: [w247 cluster{"Constellation":cdb[]}[] []] -> w186
          frame False {
          }
          frame True {
          }
        }
        "Constellation Map 2 Channel" <- w186
        "Constellation Map 1 Channel" <- w184
        n201 = local read "Switch mode"() -> (w146:bool)
        n202 = case shown="False" w153 {
          tunnel: w137 -> [w237 w241]
          tunnel: [nan ("Graph Instantaneous BER") w241] -> w143
          tunnel: [w238 T5 {"Graph Instantaneous BER"=nan, "Graph Instantaneous BER"=nan, "Graph Instantaneous BER"=nan}] -> w144
          tunnel: w136 -> [w236 _]
          tunnel: w135 -> [w235 _]
          frame False {
            n203 = Bundle("Graph Instantaneous BER"=w237, "Graph Instantaneous BER"=w236, "Graph Instantaneous BER"=w235) -> (w238:T5)  [unwired: 1 in]
          }
          frame True {
          }
        }
        "Low-Power BER - 2 Channels" <- w144
        n204 = Bundle("Graph Instantaneous BER"=w147, "Graph Instantaneous BER"=w150, "Graph Instantaneous BER"=w148) -> (w190:T5)  [unwired: 1 in]
        n205 = Equal To 0?(x="State") -> (x = 0?=w181:bool)
        "CH0 2" <- w181
        n206 = Not(x=w146) -> (.not. x?=w145:bool)
        n207 = Not(x=w181) -> (.not. x?=→"CH1 2":bool)
        n208 = case shown="True" w153 {
          tunnel: w147 -> [_ w245]
          tunnel: [nan w245] -> w189
          tunnel: w190 -> [w243 _]
          tunnel: [w243 T5 {"Graph Instantaneous BER"=nan, "Graph Instantaneous BER"=nan, "Graph Instantaneous BER"=nan}] -> w191
          frame False {
          }
          frame True {
          }
        }
        "High-Power BER" <- w191
        "High-Power BER - 1 Channel" <- w189
        n209 = case shown="False" w145 {
          tunnel: w143 -> [_ w194]
          tunnel: [w193 w194] -> w142
          frame False {
            n210 = local read "HP - CH0"() -> (w193:dbl)
          }
          frame True {
          }
        }
        "Low-Power BER - 1 Channel" <- w142
        n211 = local write "Counter"(w175) -> ()
        n212 = local write "State"(w176) -> ()
        n213 = case shown="True" w153 {
          tunnel: w137 -> [w199 w223]
          tunnel: w147 -> [w198 w222]
          tunnel: w152 -> [w201 w221]
          tunnel: ["" w219] -> w151
          tunnel: w150 -> [w197 _]
          tunnel: w148 -> [w196 _]
          tunnel: [w195 ""] -> w149
          frame False {
            n214 = case shown="True" w201 {
              tunnel: ["" w209] -> w195
              tunnel: w199 -> [_ w207]
              tunnel: w198 -> [_ w208]
              tunnel: "Save data 2 channels" -> [_ w206]
              tunnel: w197 -> [_ w205]
              tunnel: w196 -> [_ w204]
              frame False {
              }
              frame True {
                n215 = case shown="True" w206 {
                  tunnel: ["" w215] -> w209
                  tunnel: w207 -> [_ w214]
                  tunnel: w208 -> [_ w213]
                  tunnel: w205 -> [_ w212]
                  tunnel: w204 -> [_ w211]
                  frame False {
                  }
                  frame True {
                    n216 = Build Array(w214, w213, w212, w211) -> (w217:dbl[])
                    n217 = Array To Spreadsheet String(array=w217, 3:"%.3f") -> (spreadsheet string=w215:string)  [unwired: 1 out]
                  }
                }
              }
            }
          }
          frame True {
            n218 = case shown="True" w221 {
              tunnel: ["" w228] -> w219
              tunnel: w223 -> [_ w226]
              tunnel: w222 -> [_ w227]
              tunnel: "Save data 1 channel" -> [_ w225]
              frame False {
              }
              frame True {
                n219 = case shown="True" w225 {
                  tunnel: ["" w232] -> w228
                  tunnel: w226 -> [_ w231]
                  tunnel: w227 -> [_ w230]
                  frame False {
                  }
                  frame True {
                    n220 = Build Array(w231, w230) -> (w234:dbl[])
                    n221 = Array To Spreadsheet String(array=w234, 3:"%.3f") -> (spreadsheet string=w232:string)  [unwired: 1 out]
                  }
                }
              }
            }
          }
        }
      }
    }
    n222 = Write to Text File(file (use dialog)=w51, text=w46, error in=w50) -> (refnum out=w48:refnum<file>, error out=w49:errorcluster)  [unwired: 1 in, 1 out]
    n223 = Write to Text File(file (use dialog)=w57, text=w56, error in=w58) -> (refnum out=w59:refnum<file>, error out=w60:errorcluster)  [unwired: 1 in, 1 out]
    n224 = Write to Text File(file (use dialog)=w55, text=w47, error in=w53) -> (refnum out=w54:refnum<file>, error out=w52:errorcluster)  [unwired: 1 in, 1 out]
    "Numeric" <- w45
  }
  n225 = Close File(refnum=w22, error in=w23) -> (error out=w26:errorcluster)  [unwired: 1 out]
  n226 = Close File(refnum=w4, error in=w3) -> (error out=w10:errorcluster)  [unwired: 1 out]
  n227 = Close File(refnum=w2, error in=w1) -> (error out=w9:errorcluster)  [unwired: 1 out]
  n228 = local read "iterationsIM"() -> (→"iterationsIM":dbl)
  n229 = call <vilib>:"Simple Error Handler.vi"("error in (no error)"=w26) -> ()  [unwired: 1 in, 8 out]
  n230 = call <vilib>:"Simple Error Handler.vi"("error in (no error)"=w10) -> ()  [unwired: 1 in, 8 out]
  n231 = call <vilib>:"Simple Error Handler.vi"("error in (no error)"=w9) -> ()  [unwired: 1 in, 8 out]
  n232 = call <instrlib>:"niUSRP Close Session.vi"("session handle"=w36, "error in (no error)"=w37) -> ()  [unwired: 13 in, 1 out]
  "No. Bits LP - CH0" <- w33
  "No. Bits - CH1" <- w33
  "No. Bits HP - CH0" <- w33
